vi "pc.vi"() -> ()   [LabVIEW 2014]
uses:
  <vilib>/nao/NAO SDK.lvlib
panel:
  out "ErrorOut 3":errorcluster
  out "ErrorOut 2":errorcluster
  out "ErrorOut":errorcluster
  out "Numeric":i32
  in  "stop":bool
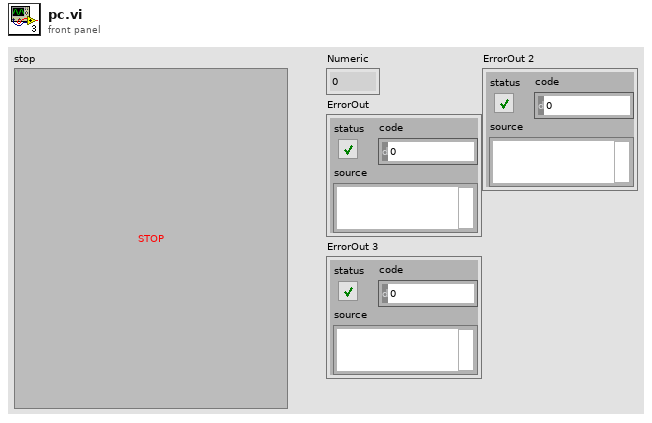
[diagram p1: front panel]
types:
  T1 = typedef "NAO SDK.lvlib/RobotPostureRef.ctl" = refnum<k1>
  T2 = typedef "NAO SDK.lvlib/BehaviorManagerRef.ctl" = refnum<k1>
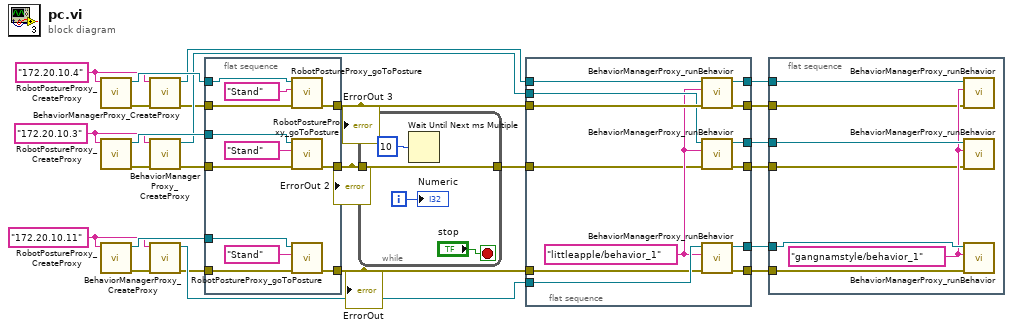
[diagram p0: block diagram]
diagram:
  w2 = "172.20.10.3" ("pIP")
  w4 = "172.20.10.4" ("pIP")
  w6 = "172.20.10.11" ("pIP")
  n1 = call <vilib>:"RobotPostureProxy_CreateProxy.vi"("pIP"=w4) -> ("ErrorOut"=w3:errorcluster, "ALPostureRef"=w24:T1)  [unwired: 9 in]
  n2 = call <vilib>:"RobotPostureProxy_CreateProxy.vi"("pIP"=w2) -> ("ErrorOut"=w1:errorcluster, "ALPostureRef"=w21:T1)  [unwired: 9 in]
  n3 = call <vilib>:"RobotPostureProxy_CreateProxy.vi"("pIP"=w6) -> ("ErrorOut"=w5:errorcluster, "ALPostureRef"=w25:T1)  [unwired: 9 in]
  n4 = call <vilib>:"BehaviorManagerProxy_CreateProxy.vi"("ErrorIn"=w3, "pIP"=w4) -> ("ErrorOut"=w16:errorcluster, "ALBehaviorRef"=w22:T2)  [unwired: 8 in]
  n5 = call <vilib>:"BehaviorManagerProxy_CreateProxy.vi"("ErrorIn"=w1, "pIP"=w2) -> ("ErrorOut"=w12:errorcluster, "ALBehaviorRef"=w18:T2)  [unwired: 8 in]
  n6 = call <vilib>:"BehaviorManagerProxy_CreateProxy.vi"("ErrorIn"=w5, "pIP"=w6) -> ("ErrorOut"=w14:errorcluster, "ALBehaviorRef"=w23:T2)  [unwired: 8 in]
  n7 = flat-sequence {
    tunnel: w25 -> [w37]
    tunnel: [w36] -> w13
    tunnel: w24 -> [w34]
    tunnel: [w33] -> w15
    tunnel: w16 -> [w31]
    tunnel: w14 -> [w30]
    tunnel: w21 -> [w28]
    tunnel: w12 -> [w27]
    tunnel: [w26] -> w11
    frame #0 {
      n8 = call <vilib>:"RobotPostureProxy_goToPosture.vi"("ErrorIn"=w31, "postureName"="Stand", "Ref"=w34) -> ("ErrorOut"=w33:errorcluster)  [unwired: 6 in, 2 out]
      n9 = call <vilib>:"RobotPostureProxy_goToPosture.vi"("ErrorIn"=w27, "postureName"="Stand", "Ref"=w28) -> ("ErrorOut"=w26:errorcluster)  [unwired: 6 in, 2 out]
      n10 = call <vilib>:"RobotPostureProxy_goToPosture.vi"("ErrorIn"=w30, "postureName"="Stand", "Ref"=w37) -> ("ErrorOut"=w36:errorcluster)  [unwired: 6 in, 2 out]
    }
  }
  n11 = while {
    tunnel: w11 -> [w41]
    tunnel: [w41] -> w10
    i -> [w38]
    stop <- "stop" stop-if-true
    n12 = Wait Until Next ms Multiple(millisecond multiple=u32 10) -> ()  [unwired: 1 out]
    "Numeric" <- w38
  }
  n13 = flat-sequence {
    tunnel: w23 -> [w54]
    tunnel: w22 -> [w53]
    tunnel: w15 -> [w52]
    tunnel: w13 -> [w51]
    tunnel: [w50] -> w20
    tunnel: [w49] -> w19
    tunnel: w18 -> [w48]
    tunnel: [w46] -> w17
    tunnel: w10 -> [w45]
    tunnel: [w44] -> w9
    tunnel: [w43] -> w8
    tunnel: [w42] -> w7
    frame #0 {
      w47 = "littleapple/behavior_1" ("name")
      n14 = call <vilib>:"BehaviorManagerProxy_runBehavior.vi"("ErrorIn"=w52, "name"=w47, "Ref"=w53) -> ("ErrorOut"=w42:errorcluster, "RefOut"=w50:T2)  [unwired: 7 in]
      n15 = call <vilib>:"BehaviorManagerProxy_runBehavior.vi"("ErrorIn"=w45, "name"=w47, "Ref"=w48) -> ("ErrorOut"=w44:errorcluster, "RefOut"=w46:T2)  [unwired: 7 in]
      n16 = call <vilib>:"BehaviorManagerProxy_runBehavior.vi"("ErrorIn"=w51, "name"=w47, "Ref"=w54) -> ("ErrorOut"=w43:errorcluster, "RefOut"=w49:T2)  [unwired: 7 in]
    }
  }
  n17 = flat-sequence {
    tunnel: w20 -> [w61]
    tunnel: w19 -> [w60]
    tunnel: w17 -> [w59]
    tunnel: w9 -> [w57]
    tunnel: w8 -> [w56]
    tunnel: w7 -> [w55]
    frame #0 {
      w58 = "gangnamstyle/behavior_1" ("name")
      n18 = call <vilib>:"BehaviorManagerProxy_runBehavior.vi"("ErrorIn"=w55, "name"=w58, "Ref"=w61) -> ()  [unwired: 7 in, 2 out]
      n19 = call <vilib>:"BehaviorManagerProxy_runBehavior.vi"("ErrorIn"=w57, "name"=w58, "Ref"=w59) -> ()  [unwired: 7 in, 2 out]
      n20 = call <vilib>:"BehaviorManagerProxy_runBehavior.vi"("ErrorIn"=w56, "name"=w58, "Ref"=w60) -> ()  [unwired: 7 in, 2 out]
    }
  }
  "ErrorOut" <- w13
  "ErrorOut 2" <- w11
  "ErrorOut 3" <- w15
